vi "Resolve (String).vi"(8 "error in (no error)":errorcluster, 10 "Element":refnum<class "Config Element.lvclass">, 11 "Sequence Constants in":refnum<class "Sequence Constants.lvclass">) -> (0 "error out":errorcluster, 2 "String Value":string, 3 "Sequence Constants out":refnum<class "Sequence Constants.lvclass">)   [LabVIEW 2020, in "VolatusSeqConfig.lvlib" / "Sequence Constants.lvclass"]
uses:
  Sequence Constants.lvclass
  lv-cdm/CDM-Config/Config Element/Config Element.lvclass
  Sequence Constants.lvclass/Sequence Constants.ctl
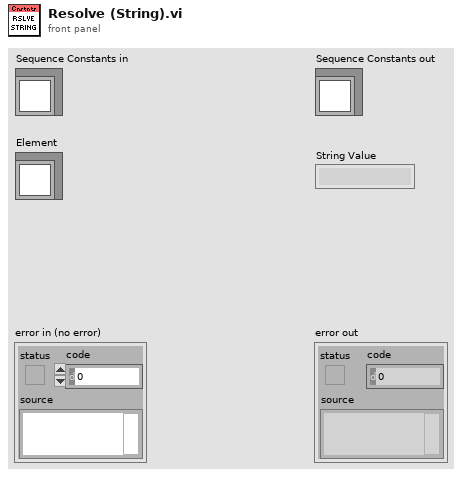
[diagram p1: front panel]
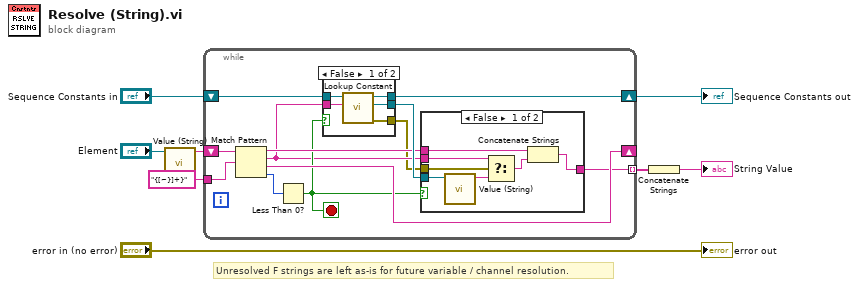
[diagram p0: block diagram]
diagram:
  # "Unresolved F strings are left as-is for future variable / channel resolution."
  n1 = call "Value (String).vi"("Config Element in"="Element") -> ("String Value"=w6:string)  [unwired: 9 in, 1 out]
  n2 = while {
    shift-right: [w14] -> _
    shift-left: w6 -> [w20]
    tunnel: "{[~}]+}" ("regular expression") -> [w19]
    shift-right: [w16] -> w4
    shift-left: "Sequence Constants in" -> [w12]
    tunnel: [w13] -> w2 mode=indexing
    stop <- w11 stop-if-true
    n3 = Match Pattern(string=w20, regular expression=w19) -> (before substring=w15:string, match substring=w10:string, after substring=w14:string, offset past match=w18:i32)  [unwired: 1 in]
    n4 = Less Than 0?(x=w18) -> (x < 0?=w11:bool)
    n5 = case shown="False" w11 {
      tunnel: w10 -> [w25 _]
      tunnel: [w24 _] -> w17
      tunnel: [w23 w26] -> w16
      tunnel: w12 -> [w22 w26]
      tunnel: [w21 _] -> w9
      frame False {
        n6 = call "Lookup Constant.vi"("Constant Name"=w25, "Sequence Constants in"=w22) -> ("error out"=w21:errorcluster, "Element"=w24:refnum<class "Config Element.lvclass">, "Sequence Constants out"=w23:refnum<class "Sequence Constants.lvclass">)  [unwired: 7 in]
      }
      frame True {
      }
    }
    n7 = case shown="False" w11 {
      tunnel: w15 -> [w32 w34]
      tunnel: w17 -> [w33 _]
      tunnel: [w31 w34] -> w13
      tunnel: w10 -> [w29 _]
      tunnel: w9 -> [w28 _]
      frame False {
        n8 = call "Value (String).vi"("Config Element in"=w33) -> ("String Value"=w30:string)  [unwired: 9 in, 1 out]
        n9 = Select(t=w29, s=w28, f=w30) -> (s? t:f=w27:string)
        n10 = Concatenate Strings(w32, w27) -> (w31:string)
      }
      frame True {
      }
    }
  }
  "Sequence Constants out" <- w4
  n11 = Concatenate Strings(w2) -> (→"String Value":string)
  "error out" <- "error in (no error)"
